vi "set_item_by_name.vi"(6 "close_item? (true)":bool=TRUE, 8 "error in (no error)":errorcluster, 9 "Item":refnum<class "Item.lvclass">, 10 "item_name":string, 11 "Table in":refnum<class "Table.lvclass">) -> (0 "error out":errorcluster, 3 "Table out":refnum<class "Table.lvclass">)   [LabVIEW 2020, in "toml_edit.lvlib" / "Table.lvclass"]
uses:
  Table.lvclass
  Item/Item.lvclass
  Table.lvclass/Table.ctl
  Item/Item.lvclass/Item.ctl
  dragon_toml_64.dll
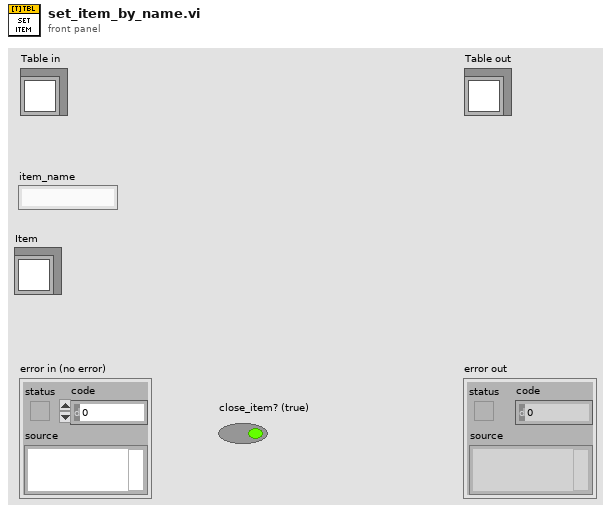
[diagram p1: front panel]
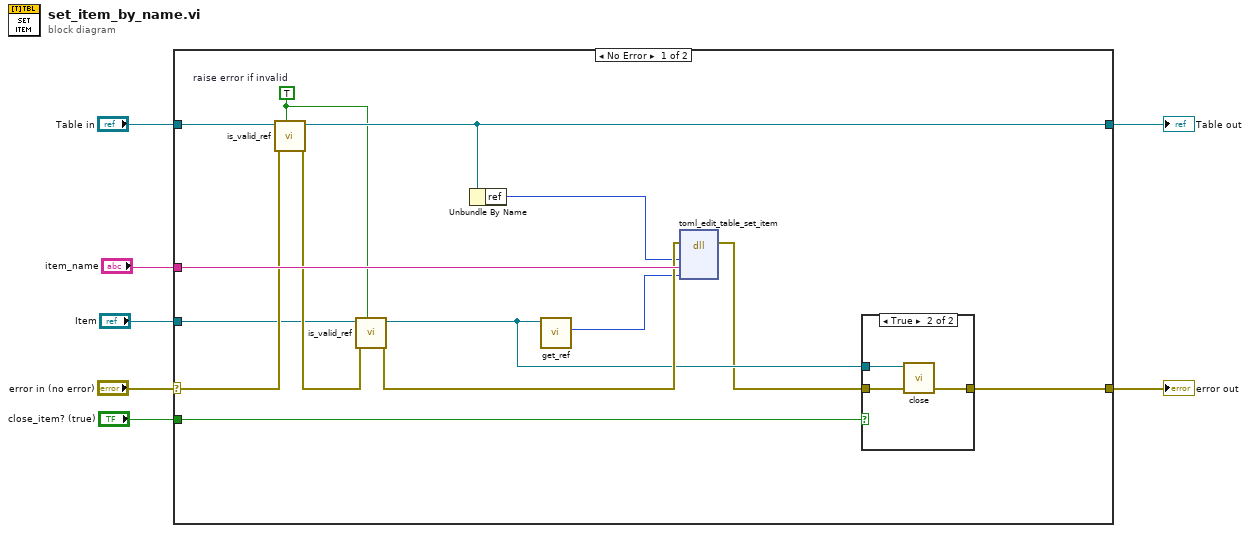
[diagram p0: block diagram]
diagram:
  n1 = case shown="No Error" "error in (no error)" {
    selector: "error in (no error)" -> [w17 w27]
    tunnel: [w20 w27] -> w6
    tunnel: [w16 w26] -> w4
    tunnel: "Table in" -> [w18 w26]
    tunnel: "item_name" -> [w21 _]
    tunnel: "Item" -> [w12 _]
    tunnel: "close_item? (true)" -> [w19 _]
    frame No Error {
      w8 = TRUE  # raise error if invalid
      n2 = call-dynamic "is_valid_ref.vi"("raise error if invalid? (False)"=w8, "error in (no error)"=w17, "Table in"=w18) -> ("error out"=w15:errorcluster, "Table out"=w16:refnum<class "Table.lvclass">)  [unwired: 6 in, 1 out]
      n3 = call-dynamic "is_valid_ref.vi"("raise error if invalid? (False)"=w8, "error in (no error)"=w15, "Item in"=w12) -> ("error out"=w14:errorcluster, "Item out"=w13:refnum<class "Item.lvclass">)  [unwired: 6 in, 1 out]
      n4 = Unbundle By Name(w16) -> ("ref"=w11:u64)
      n5 = call "get_ref.vi"("Item in"=w13) -> ("ref"=w10:u64)  [unwired: 10 in]
      n6 = dll-call lib="C:/projects/dragon-desktop/source/submodules/toml-edit-labview/lv_src/dragon_toml_*.*" fn="toml_edit_table_set_item"(error in=w14, "table_ref"=w11, "item_name"=w21, "item_ref"=w10) -> (error out=w9:errorcluster)  [unwired: 6 in, 1 out]
      n7 = case shown="True" w19 {
        tunnel: w9 -> [w22 w25]
        tunnel: [w22 w24] -> w20
        tunnel: w13 -> [_ w23]
        frame False {
        }
        frame True {
          n8 = call "close.vi"("error in (no error)"=w25, "Item in"=w23) -> ("error out"=w24:errorcluster)  [unwired: 9 in]
        }
      }
    }
    frame Error {
    }
  }
  "error out" <- w6
  "Table out" <- w4
